vi "TDMS_NewFile.vi"(8 "error in (no error)":errorcluster, 11 "Folder tmp":path) -> (0 "error out":errorcluster, 2 "Path":path, 3 "Refnum out":refnum<k34>)   [LabVIEW 2025]
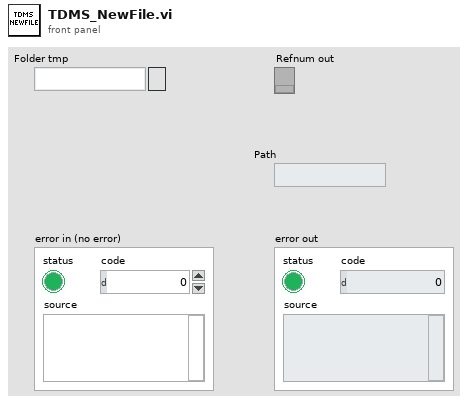
[diagram p1: front panel]
types:
  T1 = enum16{"open", "open or create", "create or replace", "create", "open (read-only)"}
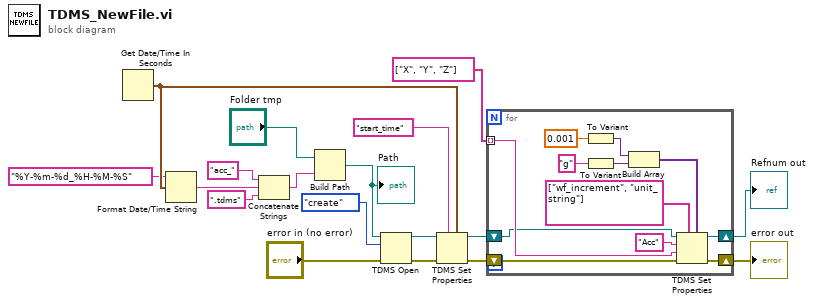
[diagram p0: block diagram]
diagram:
  n1 = Get Date/Time In Seconds() -> (seconds since 1Jan1904=w11:timestamp)
  n2 = Format Date/Time String(time format string (%c)="%Y-%m-%d_%H-%M-%S", seconds (now)=w11) -> (date/time string=w2:string)  [unwired: 1 in]
  n3 = Concatenate Strings("acc_" ("string"), w2, ".tdms" ("string")) -> (w5:string)
  n4 = Build Path(base path="Folder tmp", name or relative path=w5) -> (appended path=w7:path)
  "Path" <- w7
  n5 = TDMS Open(8:"error in (no error)", 10:T1."create" ("operation (0:open)"), 11:w7) -> (0:w9:errorcluster, 3:w14:refnum<k34>)  [unwired: 4 in]
  n6 = TDMS Set Properties(5:w11, 7:"start_time", 8:w9, 11:w14) -> (0:w16:errorcluster, 3:w15:refnum<k34>)  [unwired: 2 in, 2 out]
  n7 = for {
    tunnel: string[] ["X", "Y", "Z"] ("property names") -> [w30] mode=indexing
    shift-right: [w21] -> w17
    shift-left: w16 -> [w22]
    shift-right: [w19] -> w18
    shift-left: w15 -> [w20]
    n8 = To Variant(anything=0.001 ("number")) -> (Variant=w25:variant)
    n9 = To Variant(anything="g" ("group name")) -> (Variant=w23:variant)
    n10 = Build Array(w25, w23) -> (w28:variant[])
    n11 = TDMS Set Properties(5:w28, 7:string[] ["wf_increment", "unit_string"] ("property names"), 8:w22, 9:w30, 10:"Acc" ("group name"), 11:w20) -> (0:w21:errorcluster, 3:w19:refnum<k34>)  [unwired: 2 out]
  }
  "error out" <- w17
  "Refnum out" <- w18
